vi "Read.vi"(8 "error in (no error)":errorcluster, 11 "CTI_AnalogIn in":refnum<class "CTI_AnalogIn.lvclass">) -> (0 "error out":errorcluster, 2 "Value":T1, 3 "CTI_AnalogIn out":refnum<class "CTI_AnalogIn.lvclass">)   [LabVIEW 2021, in "CTI_AnalogIn.lvclass"]
doc: "Abstract Data Classes 2.1.1.13\nTim Streeter - TSA\nCopyright (c) 2025, TSA"
uses:
  CTI_AnalogIn.lvclass
  <vilib>/TSA/Abstract Data Classes/Abs_Types/U16 Integer/Support/Type.ctl
  CTI_AnalogIn.lvclass/CTI_AnalogIn.ctl
  <vilib>/CTI/CTI Drivers/CTI/Session/Session.lvclass
  <vilib>/TSA/Abstract Data Classes/Abs_Types/U16 Integer/Abs_U16 Integer.lvclass
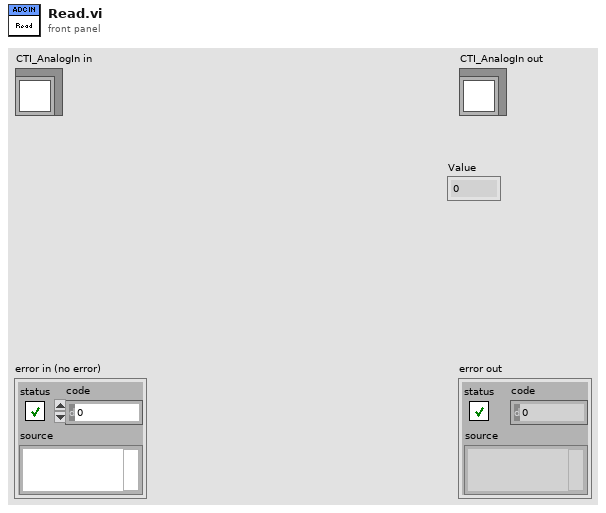
[diagram p1: front panel]
types:
  T1 = typedef "Abs_U16 Integer.lvclass/Type.ctl" = u16
  T2 = typedef "CTI.lvlib/ADC Number.ctl" = i8
  T3 = typedef "CTI.lvlib/Raw ADC.ctl" = u16
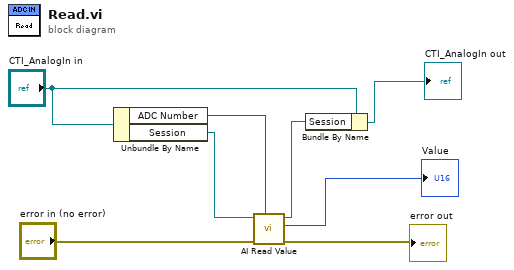
[diagram p0: block diagram]
diagram:
  n1 = Unbundle By Name("CTI_AnalogIn in") -> ("ADC Number"=w5:T2, "Session"=w4:refnum<class "Session.lvclass">)
  n2 = call <vilib>:"AI Read Value.vi"("ADC #"=w5, "error in (no error)"="error in (no error)", "Session in"=w4) -> ("error out"=→"error out":errorcluster, "Value"=→"Value":T3, "Session out"=w3:refnum<class "Session.lvclass">)  [unwired: 6 in]
  n3 = Bundle By Name(cluster="CTI_AnalogIn in", "Session"=w3) -> (→"CTI_AnalogIn out":refnum<class "CTI_AnalogIn.lvclass">)
